vi "Dmtch Get Chl Count.vi"(8 "error in (no error)":errorcluster caption="错误输入（无错误）", 11 "chlCnt":u64[](array[numeric])) -> (0 "error out":errorcluster caption="错误输出", 2 "function return":i32, 3 "chlCnt 2":u64[](array[numeric]))   [LabVIEW 2017, in "smncsftmt.lvlib"]
doc: "__declspec(dllexport) int DmtchGetChlCount(unsigned long long chlCnt[]);"
uses:
  smncsftmt.lvlib
  smncsftmt.dll
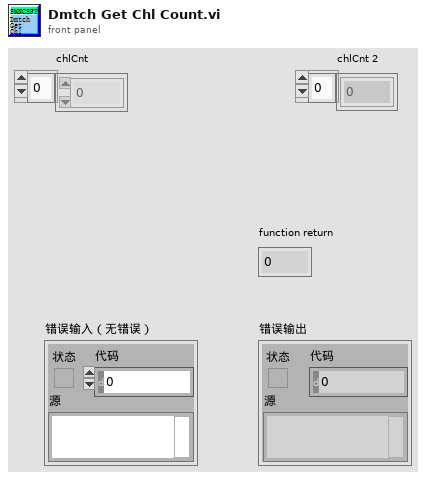
[diagram p1: front panel]
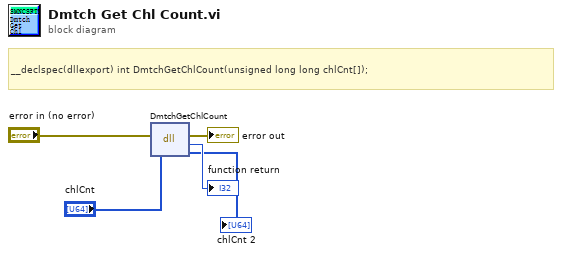
[diagram p0: block diagram]
diagram:
  # "__declspec(dllexport) int DmtchGetChlCount(unsigned long long chlCnt[]);"
  n1 = dll-call lib="PTH2oabs CUsersaDesktop\nLABVIEW范例National InstrumentsLabVIEW 2017user.lib\tsmncsftmtsmncsftmt.*" fn="DmtchGetChlCount"(error in="error in (no error)", "chlCnt"="chlCnt") -> (error out=→"error out":errorcluster, "返回类型"=→"function return":i32, "chlCnt"=→"chlCnt 2":u64[])  [unwired: 2 in, 1 out]
